vi "Filter Packets.vi"(10 "CAN Header in":T1 {"CANID and Flags" format="%.0x"; "FD Flags" format="%.0x"}, 11 "CAN_RW_CORE":refnum<class "CAN_RW_CORE.lvclass">) -> (2 "Valid":bool)   [LabVIEW 2021, in "CAN_RW_CORE.lvclass"]
uses:
  CAN_RW_CORE.lvclass
  <vilib>/CIF Foundation/CIF PCAP Parse and Build/Typedef/Socket CAN Header.ctl
  CAN_RW_CORE.lvclass/CAN_RW_CORE.ctl
  <vilib>/CIF Foundation/CIF PCAP Parse and Build/pcap_Parse_Build_CIF.lvclass
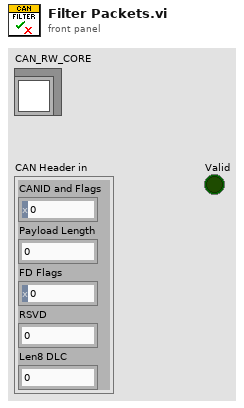
[diagram p1: front panel]
types:
  T1 = typedef "pcap_Parse_Build_CIF.lvclass/Socket CAN Header.ctl" = cluster{"CANID and Flags":u32, "Payload Length":u8, "FD Flags":u8, "RSVD":u8, "Len8 DLC":u8}
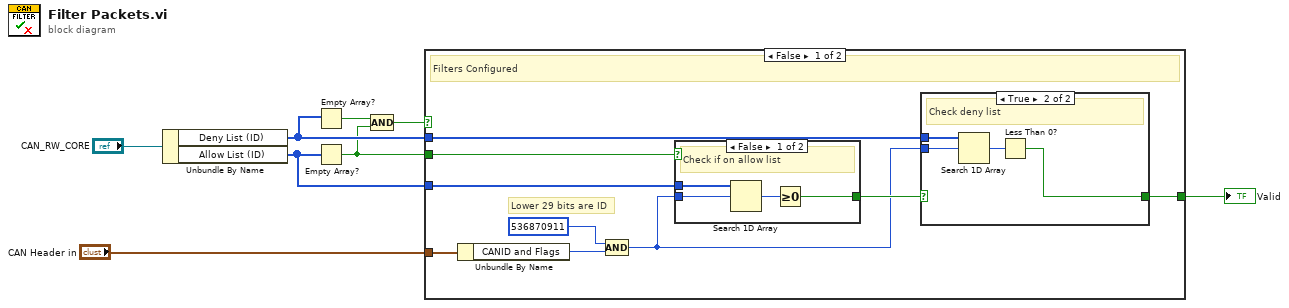
[diagram p0: block diagram]
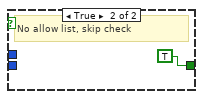
[diagram p3: hidden frame]
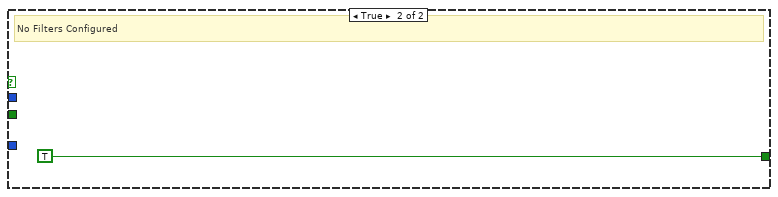
[diagram p4: hidden frame]
diagram:
  n1 = Unbundle By Name("CAN_RW_CORE") -> ("Deny List (ID)"=w6:u32[], "Allow List (ID)"=w7:u32[])
  n2 = Empty Array?(array=w6) -> (empty?=w5:bool)
  n3 = Empty Array?(array=w7) -> (empty?=w4:bool)
  n4 = Compound Arithmetic op=AND(w5, w4) -> (w3:bool)
  n5 = case shown="False" w3 {
    tunnel: w7 -> [w17 _]
    tunnel: w6 -> [w16 _]
    tunnel: w4 -> [w15 _]
    tunnel: "CAN Header in" -> [w14 _]
    tunnel: [w13 TRUE] -> w1
    frame False {
      # "Lower 29 bits are ID"
      # "Filters Configured"
      n6 = Unbundle By Name(w14) -> ("CANID and Flags"=w10:u32)
      n7 = Compound Arithmetic op=AND(u32 536870911 ("number"), w10) -> (w9:u32)
      n8 = case shown="False" w15 {
        tunnel: w17 -> [w26 _]
        tunnel: w9 -> [w25 _]
        tunnel: [w23 TRUE] -> w12
        frame False {
          # "Check if on allow list"
          n9 = Search 1D Array(1D array=w26, element=w25) -> (index of element=w24:i32)  [unwired: 1 in]
          n10 = Greater Or Equal To 0?(x=w24) -> (x >= 0?=w23:bool)
        }
        frame True {
          # "No allow list, skip check"
        }
      }
      n11 = case shown="True" w12 {
        selector: w12 -> [w18 _]
        tunnel: w16 -> [_ w22]
        tunnel: w9 -> [_ w21]
        tunnel: [w18 w19] -> w13
        frame False {
          # "Failed allow list check, skip."
        }
        frame True {
          # "Check deny list"
          n12 = Search 1D Array(1D array=w22, element=w21) -> (index of element=w20:i32)  [unwired: 1 in]
          n13 = Less Than 0?(x=w20) -> (x < 0?=w19:bool)
        }
      }
    }
    frame True {
      # "No Filters Configured"
    }
  }
  "Valid" <- w1
